vi "SC Project Menu.vi"(9 "projects":T1(array[cluster]), 10 "selected":i32, 11 "position":cluster{"Left":i32, "Top":i32, "Width":i32}={"Left"=400, "Top"=300, "Width"=200}) -> (1 "index":i32=-1)   [LabVIEW 2023]
doc: "A drop-down list of the robot's projects in its own borderless window, over the ring it drops from: position (screen coordinates) is that ring's top left and width. The window shows a copy of the ring (the selected project) with the list just below it, like the ring's own list. The list is in name order (index still refers to projects); bold marks the project the robot runs, italics one without a local copy on this computer. Clicking a project (pressed in the list, or dragged onto another project) or Return returns its index; clicking the ring again, Escape or moving the mouse out (other than from the list into the ring) returns -1."
panel:
  in  "Field":u16(ring)
  in  "Projects":i32(listbox)=-1
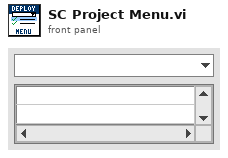
[diagram p1: front panel]
types:
  T1 = cluster{"name":string, "running":bool, "local copy":bool}[]
  T2 = cluster{"name":string, "running":bool, "local copy":bool}
  T3 = typedef "LVPositionTypeDef.ctl" = cluster{"Left":i32, "Top":i32}
  T4 = typedef "LVPoint32TypeDef.ctl" = cluster{"Horizontal":i32, "Vertical":i32}
  T5 = typedef "LVRowAndColumnTypeDef.ctl" = cluster{"Row":i32, "Column":i32}
  T6 = typedef "eventvkey.ctl" = enum16{"ASCII", "Enter", "Return", "Shift", "Ctrl", "Alt", "Cmd", "Opt", "Caps", "NumLock", "Clear", "Break", "Up", "Down", "Left", "Right", "Insert", "Delete", "Home", "End", "PageUp", "PageDown", "Escape", "Help", "Pause", "ScrollLock", "F1", "F2", "F3", "F4", "F5", "F6", "F7", "F8", "F9", "F10", "F11", "F12", "F13", "F14", "F15", "F16", "F17", "F18", "F19", "F20", "F21", "F22", "F23", "F24", "Play", "VolumeUp", "VolumeDown", "Mute", "Two Byte Char"}
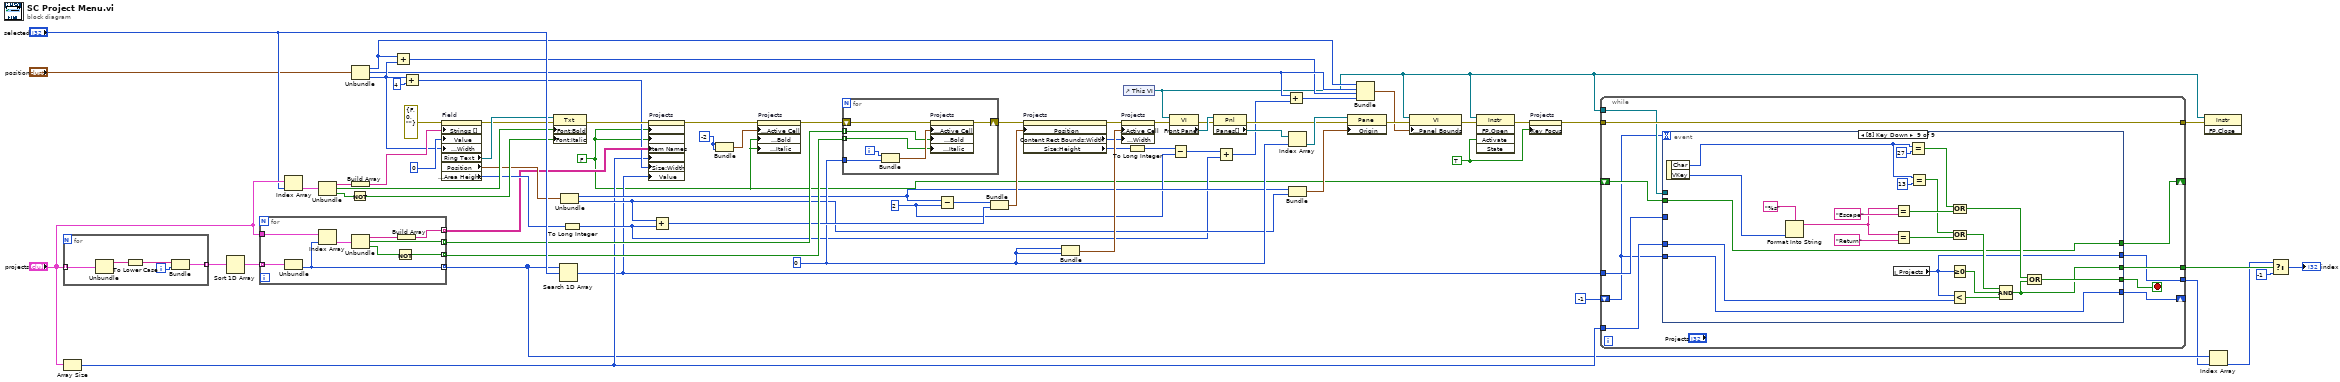
[diagram p0: block diagram]
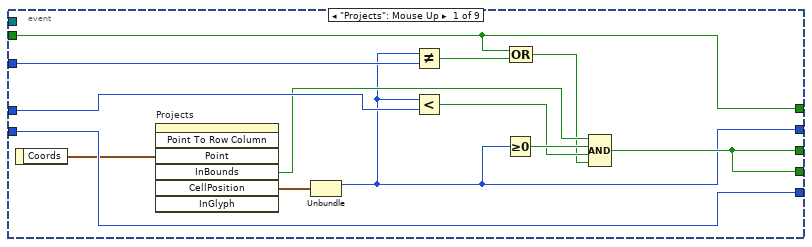
[diagram p2: hidden frame]
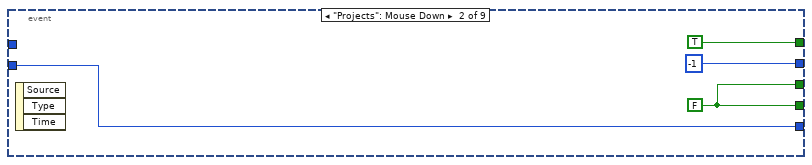
[diagram p3: hidden frame]
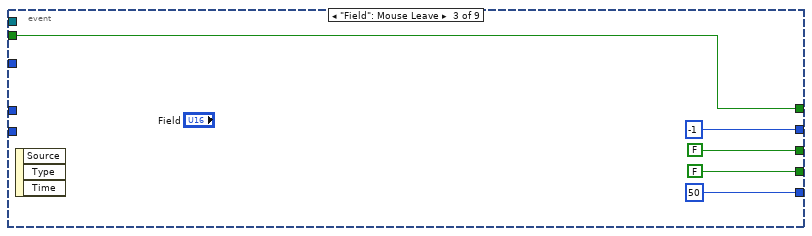
[diagram p4: hidden frame]
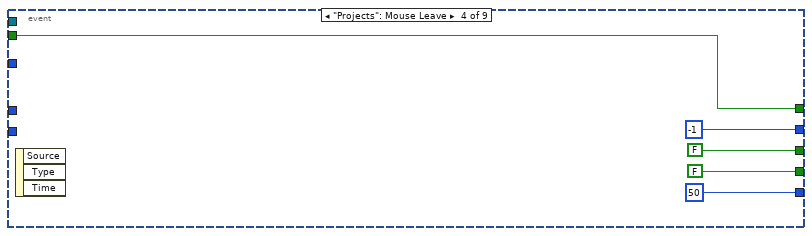
[diagram p5: hidden frame]
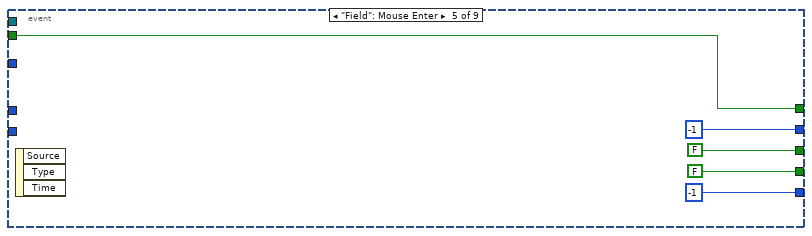
[diagram p6: hidden frame]
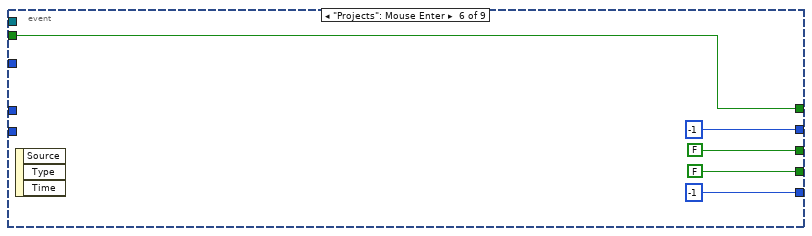
[diagram p7: hidden frame]
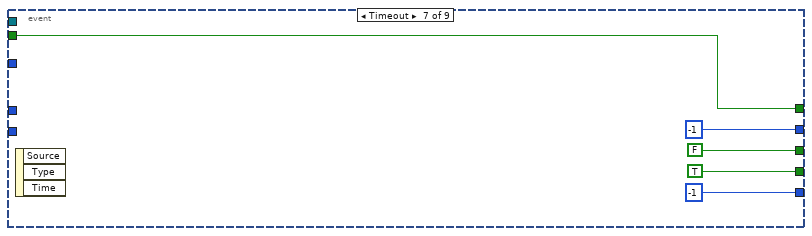
[diagram p8: hidden frame]
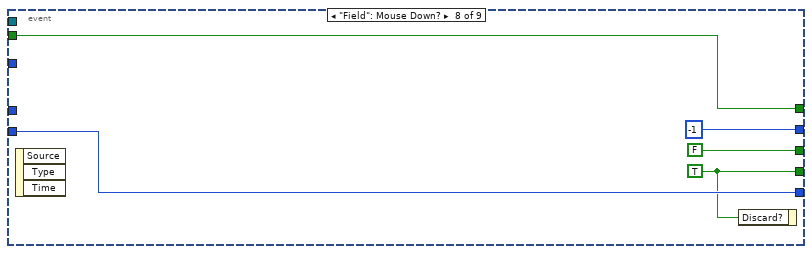
[diagram p9: hidden frame]
diagram:
  w26 = 2
  w14 = TRUE
  w9 = FALSE
  w52 = -2
  w35 = 0
  n1 = for {
    tunnel: "projects" -> [w78] mode=indexing
    tunnel: [w75] -> w73 mode=indexing
    i -> [w74]
    n2 = Unbundle(w78) -> ("name"=w77:string)  [unwired: 2 out]
    n3 = To Lower Case(string=w77) -> (all lower case string=w76:string)
    n4 = Bundle(w76, w74) -> (w75:cluster{string, i32})  [unwired: 1 in]
  }
  n5 = Array Size(array="projects") -> (size(s)=w13:i32)
  n6 = Sort 1D Array(array=w73) -> (sorted array=w72:cluster{string, i32}[])
  n7 = for {
    tunnel: w72 -> [w87] mode=indexing
    tunnel: "projects" -> [w86]
    tunnel: [w85] -> w8 mode=indexing
    tunnel: [w81] -> w54 mode=indexing
    tunnel: [w80] -> w49 mode=indexing
    tunnel: [w79] -> w48 mode=indexing
    n8 = Unbundle(w87) -> (w85:i32)  [unwired: 1 out]
    n9 = Index Array(array=w86, index=w85) -> (element=w84:T2)
    n10 = Unbundle(w84) -> ("name"=w83:string, "running"=w80:bool, "local copy"=w82:bool)
    n11 = Not(x=w82) -> (.not. x?=w79:bool)
    n12 = Build Array(w83) -> (w81:string[])
  }
  n13 = Index Array(array="projects", index="selected") -> (element=w69:T2)
  n14 = Unbundle(w69) -> ("name"=w68:string, "running"=w61:bool, "local copy"=w67:bool)
  n15 = Not(x=w67) -> (.not. x?=w60:bool)
  n16 = Unbundle("position") -> ("Left"=w22:i32, "Top"=w21:i32, "Width"=w28:i32)
  n17 = Build Array(w68) -> (w65:string[])
  n18 = Add(x=w22, y=w28) -> (x+y=w20:i32)
  n19 = Add(x=w28, y=4) -> (x+y=w53:i32)
  n20 = property on="Field" class="Ring (strict)"(error in=errorcluster {"status"=FALSE, "code"=0, "source"=""}, "Strings []"=w65, "Value"=u16 0, "Named Numeric Size:Width"=w28) -> (error out=w62:errorcluster, "Ring Text"=w63:refnum<vi>, "Position"=w59:T3, "Bounds:Area Height"=w58:u32)  [unwired: 1 in, 1 out]
  n21 = property class="Txt"(reference=w63, error in=w62, "Font:Bold"=w61, "Font:Italic"=w60) -> (error out=w55:errorcluster)  [unwired: 1 out]
  n22 = Search 1D Array(1D array=w8, element="selected") -> (index of element=w11:i32)  [unwired: 1 in]
  n23 = Unbundle(w59) -> ("Left"=w34:i32, "Top"=w33:i32)
  n24 = To Long Integer(number=w58) -> (32bit integer=w24:i32)
  n25 = property on="Projects" class="MCListbox (strict)"(error in=w55, "Visible Items:Vertical Scrollbar Visible"=w9, "Visible Items:Horizontal Scrollbar Visible"=w9, "Item Names"=w54, "Number of Rows"=w13, "Size:Width"=w53, "Value"=w11) -> (error out=w51:errorcluster)  [unwired: 1 in, 1 out]
  n26 = Add(x=w33, y=w24) -> (x+y=w45:i32)
  n27 = Bundle(w52, w52) -> (w50:cluster{i32, i32})  [unwired: 1 in]
  n28 = property on="Projects" class="MCListbox (strict)"(error in=w51, "Active Cell:Active Cell"=w50, "Active Cell:Cell Font:Bold"=w9, "Active Cell:Cell Font:Italic"=w9) -> (error out=w47:errorcluster)  [unwired: 1 in, 1 out]
  n29 = for {
    tunnel: w49 -> [w91] mode=indexing
    tunnel: w48 -> [w90] mode=indexing
    tunnel: w35 -> [w94]
    shift-right: [w89] -> w44
    shift-left: w47 -> [w93]
    i -> [w88]
    n30 = Bundle(w88, w94) -> (w92:cluster{i32, i32})  [unwired: 1 in]
    n31 = property on="Projects" class="MCListbox (strict)"(error in=w93, "Active Cell:Active Cell"=w92, "Active Cell:Cell Font:Bold"=w91, "Active Cell:Cell Font:Italic"=w90) -> (error out=w89:errorcluster)  [unwired: 1 in, 1 out]
  }
  n32 = Subtract(x=w34, y=w26) -> (x-y=w46:i32)
  n33 = Bundle(w46, w45) -> (w43:cluster{i32, i32})  [unwired: 1 in]
  n34 = property on="Projects" class="MCListbox (strict)"(error in=w44, "Position"=w43) -> (error out=w42:errorcluster, "Content Rect Bounds:Width"=w40:i32, "Size:Height"=w29:u32)  [unwired: 1 in, 1 out]
  n35 = Bundle(w35, w35) -> (w41:cluster{i32, i32})  [unwired: 1 in]
  n36 = property on="Projects" class="MCListbox (strict)"(error in=w42, "Active Cell:Active Cell"=w41, "Active Cell:Cell Size:Width"=w40) -> (error out=w39:errorcluster)  [unwired: 1 in, 1 out]
  n37 = control-ref of="This VI"() -> (w2:refnum<vi>)
  n38 = To Long Integer(number=w29) -> (32bit integer=w27:i32)
  n39 = property class="VI"(reference=w2, error in=w39) -> (error out=w37:errorcluster, "Front Panel"=w38:refnum<vi>)  [unwired: 1 out]
  n40 = Subtract(x=w27, y=w26) -> (x-y=w25:i32)
  n41 = property class="Pnl"(reference=w38, error in=w37) -> (error out=w31:errorcluster, "Panes[]"=w36:refnum<vi>[])  [unwired: 1 out]
  n42 = Add(x=w25, y=w24) -> (x+y=w23:i32)
  n43 = Add(x=w21, y=w23) -> (x+y=w19:i32)
  n44 = Index Array(array=w36, index=w35) -> (element=w32:refnum<vi>)
  n45 = Bundle("Left"=w34, "Top"=w33) -> (w30:cluster{"Left":i32, "Top":i32})  [unwired: 1 in]
  n46 = property class="Pane"(reference=w32, error in=w31, "Origin"=w30) -> (error out=w18:errorcluster)  [unwired: 1 out]
  n47 = Bundle("Left"=w22, "Top"=w21, w20, w19) -> (w17:cluster{"Left":i32, "Top":i32, i32, i32})  [unwired: 1 in]
  n48 = property class="VI"(reference=w2, error in=w18, "Front Panel Window:Panel Bounds"=w17) -> (error out=w16:errorcluster)  [unwired: 1 out]
  n49 = invoke class="Instr" method="FP.Open"(reference=w2, error in=w16, "Activate"=w14) -> (error out=w15:errorcluster)  [unwired: 2 in, 4 out]
  n50 = property on="Projects" class="MCListbox (strict)"(error in=w15, "Key Focus"=w14) -> (error out=w12:errorcluster)  [unwired: 1 in, 1 out]
  n51 = while {
    tunnel: w13 -> [w104]
    tunnel: w2 -> [w103]
    tunnel: w12 -> [w105]
    tunnel: w11 -> [w100]
    shift-right: [w97] -> _
    shift-left: -1 -> [w95]
    shift-right: [w98] -> _
    shift-left: w9 -> [w99]
    tunnel: [w102] -> w6
    tunnel: [w101] -> w7
    tunnel: [w105] -> w1
    stop <- w96 stop-if-true
    n52 = event shown="[8] Key Down" {
      selector: _ -> [_ _ _ _ _ _ _ _ _]
      dyn-events: _ -> [_ _ _ _ _ _ _ _ _]
      timeout: w95 -> [_ _ _ _ _ _ _ _ _]
      tunnel: w104 -> [w117 _ _ _ _ _ _ _ w168]
      tunnel: w103 -> [_ _ _ _ _ _ _ _ _]
      tunnel: [w110 w122 FALSE FALSE FALSE FALSE TRUE w148 w159] -> w96
      tunnel: [w110 w122 FALSE FALSE FALSE FALSE FALSE FALSE w158] -> w102
      tunnel: [w109 -1 -1 -1 -1 -1 -1 -1 w157] -> w101
      tunnel: w100 -> [w116 _ _ _ _ _ _ _ _]
      tunnel: w99 -> [w108 _ w124 w129 w134 w139 w144 w150 w156]
      tunnel: [w108 TRUE w124 w129 w134 w139 w144 w150 w156] -> w98
      tunnel: w95 -> [w107 w119 _ _ _ _ _ w149 w155]
      tunnel: [w107 w119 50 50 -1 -1 -1 w149 w155] -> w97
      event "Projects": Mouse Up {
        n53 = event-data() -> ("Coords"=w106:T4)  [unwired: 1 in]
        n54 = invoke on="Projects" class="MCListbox (strict)" method="Point To Row Column"("Point"=w106) -> ("InBounds"=w114:bool, "CellPosition"=w118:T5)  [unwired: 6 in, 5 out]
        n55 = Unbundle(w118) -> ("Row"=w109:i32)  [unwired: 1 out]
        n56 = Not Equal?(x=w109, y=w116) -> (x != y?=w115:bool)
        n57 = Less?(x=w109, y=w117) -> (x < y?=w112:bool)
        n58 = Greater Or Equal To 0?(x=w109) -> (x >= 0?=w113:bool)
        n59 = Compound Arithmetic op=OR(w108, w115) -> (w111:bool)
        n60 = Compound Arithmetic op=AND(w114, w113, w112, w111) -> (w110:bool)
      }
      event "Projects": Mouse Down {
        w122 = FALSE
        n61 = event-data() -> ()  [unwired: 1 in, 3 out]
      }
      event "Field": Mouse Leave {
        n62 = event-data() -> ()  [unwired: 1 in, 3 out]
      }
      event "Projects": Mouse Leave {
        n63 = event-data() -> ()  [unwired: 1 in, 3 out]
      }
      event "Field": Mouse Enter {
        n64 = event-data() -> ()  [unwired: 1 in, 3 out]
      }
      event "Projects": Mouse Enter {
        n65 = event-data() -> ()  [unwired: 1 in, 3 out]
      }
      event Timeout {
        n66 = event-data() -> ()  [unwired: 1 in, 3 out]
      }
      event "Field": Mouse Down? {
        w148 = TRUE
        n67 = event-data() -> ()  [unwired: 1 in, 3 out]
        n68 = event-data("Discard?"=w148) -> ()  [unwired: 1 in, 1 out]
      }
      event Key Down {
        n69 = event-data() -> ("Char"=w154:i16, "VKey"=w153:T6)  [unwired: 1 in]
        n70 = Format Into String(format string="%s", w153) -> (resulting string=w172:string)  [unwired: 2 in, 1 out]
        n71 = local read "Projects"() -> (w157:i32)
        n72 = Equal?(x=w172, y="Escape") -> (x = y?=w166:bool)
        n73 = Equal?(x=w172, y="Return") -> (x = y?=w164:bool)
        n74 = Equal?(x=w154, y=27) -> (x = y?=w167:bool)
        n75 = Equal?(x=w154, y=13) -> (x = y?=w165:bool)
        n76 = Greater Or Equal To 0?(x=w157) -> (x >= 0?=w162:bool)
        n77 = Less?(x=w157, y=w168) -> (x < y?=w161:bool)
        n78 = Compound Arithmetic op=OR(w167, w166) -> (w160:bool)
        n79 = Compound Arithmetic op=OR(w165, w164) -> (w163:bool)
        n80 = Compound Arithmetic op=AND(w163, w162, w161) -> (w158:bool)
        n81 = Compound Arithmetic op=OR(w160, w158) -> (w159:bool)
      }
    }
  }
  n82 = invoke class="Instr" method="FP.Close"(reference=w2, error in=w1) -> ()  [unwired: 1 in, 3 out]
  n83 = Index Array(array=w8, index=w7) -> (element=w5:i32)
  n84 = Select(t=w5, s=w6, f=-1) -> (s? t:f=→"index":i32)
